vi "NR Handover.vi"(8 "error in (no error)":errorcluster caption="에러 입력(에러 없음)", 10 "NR Call Handover Param":T1, 11 "Instrument Manager 입력":refnum<class "Instrument Manager.lvclass">) -> (0 "error out":errorcluster caption="에러 출력", 3 "Instrument Manager 출력":refnum<class "Instrument Manager.lvclass">)   [LabVIEW 2023, in "Instrument Manager.lvclass"]
uses:
  Instrument Manager.lvclass
  Type Definition/NR Handover Param.ctl
  Module/ANRITSU Call Box/Type Definition/NR Modulation Type.ctl
  6beca21e-8a86-4599-8fdc-efac4d8e6348.vi
  1c1796af-5488-416f-b3e7-f2865a0be64d.vi
  44b1f486-885c-4af6-9b29-c4b0bf21b9b9.vi
  737233f4-6f10-4002-8906-c67257dda749.vi
  8d30c4ba-745f-4322-9b4d-9fdc41ae9ab7.vi
  Instrument Manager.lvclass/Instrument Manager.ctl
  Module/ANRITSU Call Box/ANRITSU Call Box.lvlib
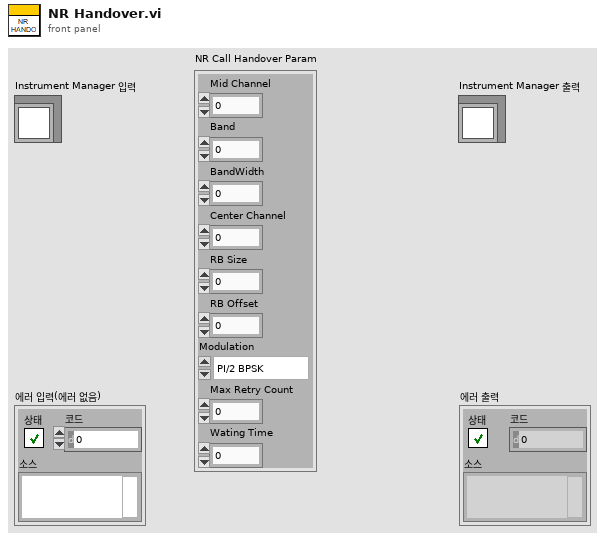
[diagram p1: front panel]
types:
  T1 = typedef "NR Handover Param.ctl" = cluster{"Mid Channel":u32, "Band":u32, "BandWidth":u32, "Center Channel":u32, "RB Size":i32, "RB Offset":i32, "Modulation":T2, "Max Retry Count":i32, "Wating Time":i32}
  T2 = typedef "ANRITSU Call Box.lvlib/NR Modulation Type.ctl" = enum16{"PI/2 BPSK", "QPSK", "16QAM", "64QAM", "256QAM"}
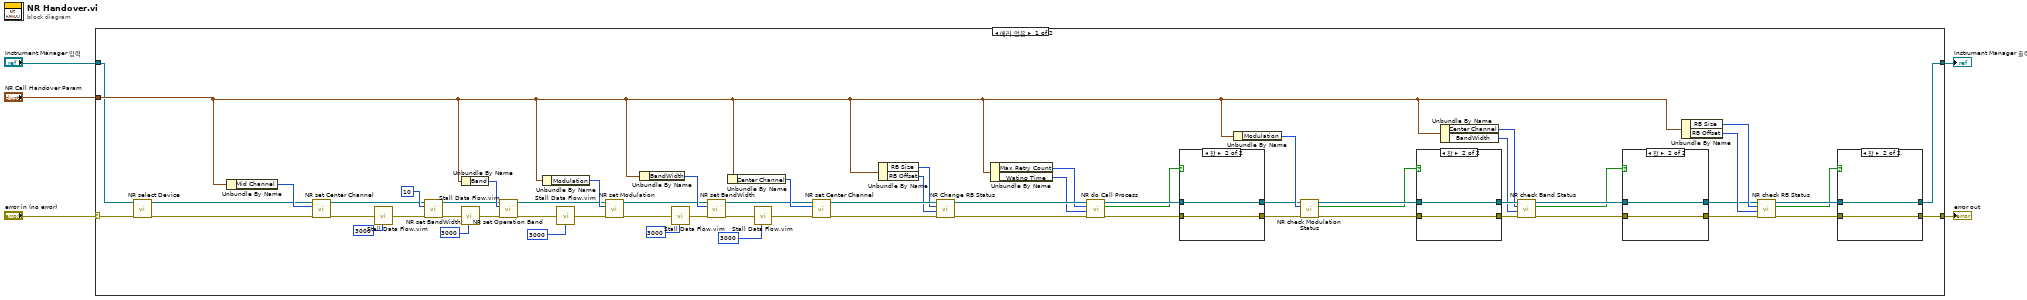
[diagram p0: block diagram]
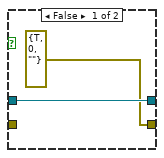
[diagram p2: hidden frame]
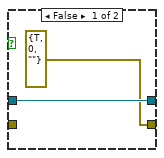
[diagram p3: hidden frame]
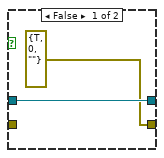
[diagram p4: hidden frame]
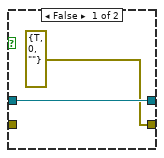
[diagram p5: hidden frame]
diagram:
  n1 = case shown="에러 없음" "error in (no error)" {
    selector: "error in (no error)" -> [w9 w87]
    tunnel: [w58 w87] -> w4
    tunnel: [w57 w86] -> w2
    tunnel: "Instrument Manager 입력" -> [w6 w86]
    tunnel: "NR Call Handover Param" -> [w12 _]
    frame No Error {
      n2 = call "NR select Device.vi"("error in (no error)"=w9, "Instrument Manager 입력"=w6) -> ("error out"=w8:errorcluster, "Instrument Manager 출력"=w7:refnum<class "Instrument Manager.lvclass">)  [unwired: 8 in]
      n3 = Unbundle By Name(w12) -> ("Mid Channel"=w51:u32)
      n4 = call "NR set Center Channel.vi"("error in (no error)"=w8, "Center Channel Number"=w51, "Instrument Manager 입력"=w7) -> ("error out"=w44:errorcluster, "Instrument Manager 출력"=w49:refnum<class "Instrument Manager.lvclass">)  [unwired: 7 in]
      n5 = call "Stall Data Flow.vim"("value in"=w44, "milliseconds to wait"=u32 3000 ("millisecond timer value")) -> ("value out"=w43:errorcluster)  [unwired: 1 out]
      n6 = call "NR set BandWidth.vi"("error in (no error)"=w43, "BW (MHz)"=u32 10, "Instrument Manager 입력"=w49) -> ("error out"=w41:errorcluster, "Instrument Manager 출력"=w47:refnum<class "Instrument Manager.lvclass">)  [unwired: 7 in]
      n7 = Unbundle By Name(w12) -> ("Band"=w48:u32)
      n8 = call "Stall Data Flow.vim"("value in"=w41, "milliseconds to wait"=u32 3000 ("millisecond timer value")) -> ("value out"=w40:errorcluster)  [unwired: 1 out]
      n9 = call "NR set Operation Band.vi"("error in (no error)"=w40, "Operation Band"=w48, "Instrument Manager 입력"=w47) -> ("error out"=w14:errorcluster, "Instrument Manager 출력"=w15:refnum<class "Instrument Manager.lvclass">)  [unwired: 7 in]
      n10 = Unbundle By Name(w12) -> ("Modulation"=w18:T2)
      n11 = call "Stall Data Flow.vim"("value in"=w14, "milliseconds to wait"=u32 3000 ("millisecond timer value")) -> ("value out"=w13:errorcluster)  [unwired: 1 out]
      n12 = call "NR set Modulation.vi"("error in (no error)"=w13, "Modulation"=w18, "Instrument Manager 입력"=w15) -> ("error out"=w17:errorcluster, "Instrument Manager 출력"=w16:refnum<class "Instrument Manager.lvclass">)  [unwired: 7 in]
      n13 = Unbundle By Name(w12) -> ("BandWidth"=w46:u32)
      n14 = call "Stall Data Flow.vim"("value in"=w17, "milliseconds to wait"=u32 3000 ("millisecond timer value")) -> ("value out"=w38:errorcluster)  [unwired: 1 out]
      n15 = call "NR set BandWidth.vi"("error in (no error)"=w38, "BW (MHz)"=w46, "Instrument Manager 입력"=w16) -> ("error out"=w20:errorcluster, "Instrument Manager 출력"=w19:refnum<class "Instrument Manager.lvclass">)  [unwired: 7 in]
      n16 = Unbundle By Name(w12) -> ("Center Channel"=w34:u32)
      n17 = call "Stall Data Flow.vim"("value in"=w20, "milliseconds to wait"=u32 3000 ("millisecond timer value")) -> ("value out"=w35:errorcluster)  [unwired: 1 out]
      n18 = call "NR set Center Channel.vi"("error in (no error)"=w35, "Center Channel Number"=w34, "Instrument Manager 입력"=w19) -> ("error out"=w32:errorcluster, "Instrument Manager 출력"=w33:refnum<class "Instrument Manager.lvclass">)  [unwired: 7 in]
      n19 = Unbundle By Name(w12) -> ("RB Size"=w31:i32, "RB Offset"=w30:i32)
      n20 = call "NR Change RB Status.vi"("error in (no error)"=w32, "RB Offset"=w30, "RB Size"=w31, "Instrument Manager 입력"=w33) -> ("error out"=w25:errorcluster, "Instrument Manager 출력"=w23:refnum<class "Instrument Manager.lvclass">)  [unwired: 6 in]
      n21 = Unbundle By Name(w12) -> ("Max Retry Count"=w10:i32, "Wating Time"=w11:i32)
      n22 = call "NR do Call Process.vi"("error in (no error)"=w25, "Waiting Time"=w11, "Max Retry Count"=w10, "Instrument Manager 입력"=w23) -> ("error out"=w24:errorcluster, "Connected?"=w21:bool, "Instrument Manager 출력"=w22:refnum<class "Instrument Manager.lvclass">)  [unwired: 5 in]
      n23 = case shown="참" w21 {
        tunnel: w22 -> [w71 w73]
        tunnel: [w71 w73] -> w27
        tunnel: [errorcluster {"status"=TRUE, "code"=0, "source"=""} ("error out") w72] -> w26
        tunnel: w24 -> [_ w72]
        frame False {
        }
        frame True {
        }
      }
      n24 = Unbundle By Name(w12) -> ("Modulation"=w56:T2)
      n25 = call "NR check Modulation Status.vi"("error in (no error)"=w26, "Modulation"=w56, "Instrument Manager 입력"=w27) -> ("error out"=w68:errorcluster, "Success?"=w63:bool, "Instrument Manager 출력"=w69:refnum<class "Instrument Manager.lvclass">)  [unwired: 6 in]
      n26 = case shown="참" w63 {
        tunnel: w69 -> [w83 w85]
        tunnel: [w83 w85] -> w67
        tunnel: [errorcluster {"status"=TRUE, "code"=0, "source"=""} ("error out") w84] -> w66
        tunnel: w68 -> [_ w84]
        frame False {
        }
        frame True {
        }
      }
      n27 = Unbundle By Name(w12) -> ("Center Channel"=w54:u32, "BandWidth"=w55:u32)
      n28 = call "NR check Band Status.vi"("error in (no error)"=w66, "BW (MHz)"=w55, "Center Channel Number"=w54, "Instrument Manager 입력"=w67) -> ("error out"=w65:errorcluster, "Success?"=w62:bool, "Instrument Manager 출력"=w64:refnum<class "Instrument Manager.lvclass">)  [unwired: 5 in]
      n29 = case shown="참" w62 {
        tunnel: w64 -> [w79 w81]
        tunnel: [w79 w81] -> w29
        tunnel: [errorcluster {"status"=TRUE, "code"=0, "source"=""} ("error out") w80] -> w28
        tunnel: w65 -> [_ w80]
        frame False {
        }
        frame True {
        }
      }
      n30 = Unbundle By Name(w12) -> ("RB Size"=w52:i32, "RB Offset"=w53:i32)
      n31 = call "NR check RB Status.vi"("error in (no error)"=w28, "RB Offset"=w53, "RB Size"=w52, "Instrument Manager 입력"=w29) -> ("error out"=w60:errorcluster, "Success?"=w59:bool, "Instrument Manager 출력"=w61:refnum<class "Instrument Manager.lvclass">)  [unwired: 5 in]
      n32 = case shown="참" w59 {
        tunnel: w61 -> [w75 w77]
        tunnel: [w75 w77] -> w57
        tunnel: [errorcluster {"status"=TRUE, "code"=0, "source"=""} ("error out") w76] -> w58
        tunnel: w60 -> [_ w76]
        frame False {
        }
        frame True {
        }
      }
    }
    frame Error {
    }
  }
  "error out" <- w4
  "Instrument Manager 출력" <- w2
